vi "Condition_Compare.vi"(8 "error in (no error)":errorcluster={"status"=FALSE, "code"=0, "source"="\"\""}, 10 "operator":string, 11 "Typed operands":string) -> (0 "error out":errorcluster={"status"=FALSE, "code"=0, "source"="\"\""}, 2 "status ok":bool, 3 "ConditionResult":string)   [LabVIEW 2026]
doc: "INTENT: Evaluate typed comparison leaf. LOGIC: Resolve both operands, convert compatible units, compare in-range/greater/equal/relative tolerance."
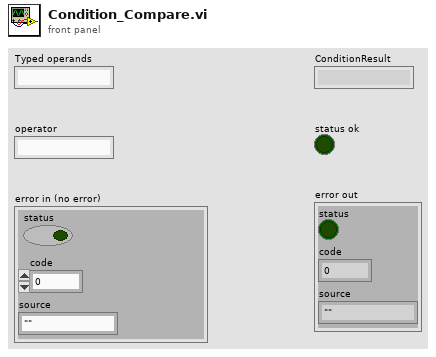
[diagram p1: front panel]
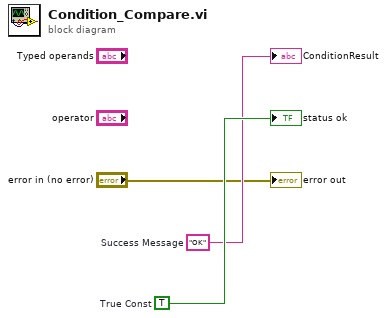
[diagram p0: block diagram]
diagram:
  w3 = TRUE  # True Const
  w2 = "OK"  # Success Message
  "ConditionResult" <- w2
  "status ok" <- w3
  "error out" <- "error in (no error)"
